vi "SelDataTbl (SubVI).vi"(8 "error in (no error)":errorcluster, 10 "In":dbl[][](array[numeric]), 11 "Enum":T1(ring)) -> (0 "error out":errorcluster, 3 "Out":dbl[][](array[numeric]))   [LabVIEW 2017]
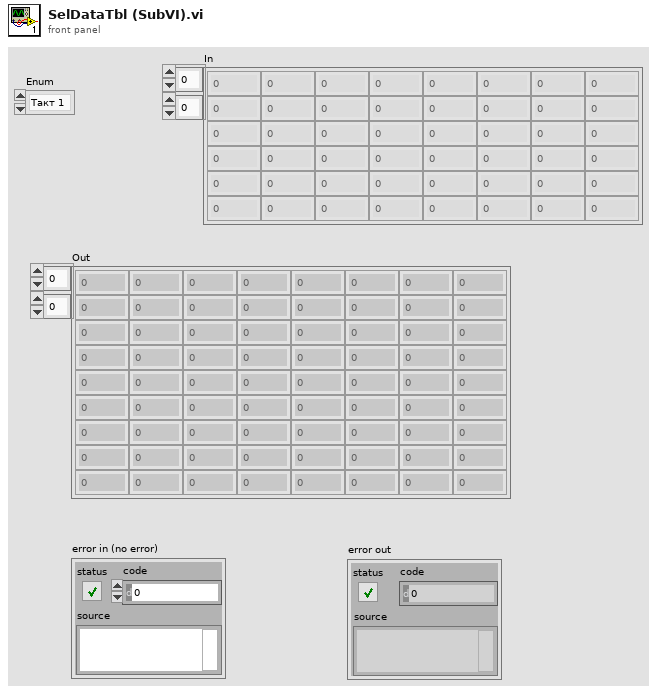
[diagram p1: front panel]
types:
  T1 = enum16{"Такт 1", "Такт 2", "Такт 3", "Такт 4", "Такт 5", "Такт 6", "Такт 7", "Такт 8", "Такт 9", "Такт 10", "Такт 11", "Такт 12", "Такт 13", "Такт 14", "Такт 15", "Такт 16", "Такт 17", "Такт 18", "Такт 19", "Такт 20", "Такт 21", "Такт 22", "Такт 23", "Такт 24", "Такт 25", "Такт 26", "Такт 27", "Такт 28", "Такт 29", "Такт 30", "Такт 31", "Такт 32"}
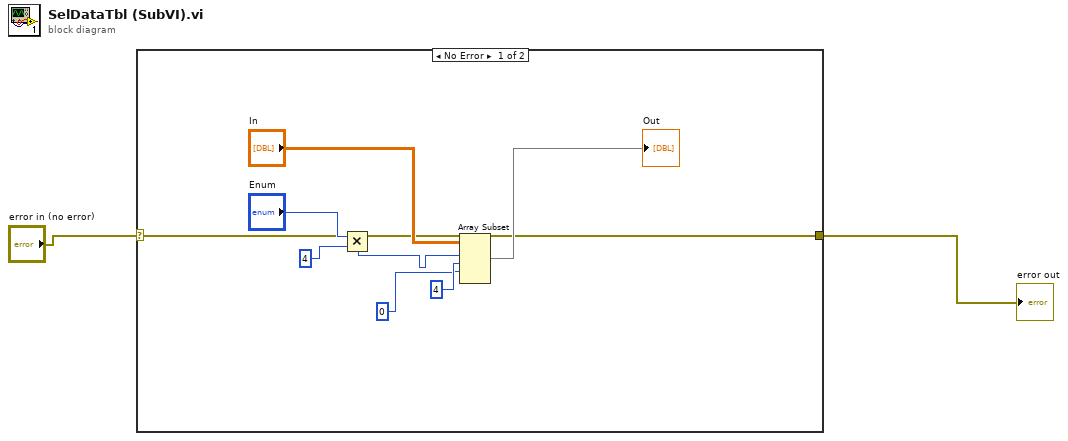
[diagram p0: block diagram]
diagram:
  n1 = case shown="No Error" "error in (no error)" {
    selector: "error in (no error)" -> [w3 w11]
    tunnel: [w3 w11] -> w1
    frame No Error {
      n2 = Multiply(x="Enum", y=4) -> (x*y=w5:i32)
      n3 = Array Subset(array="In", index (row)=w5, length (row)=4 ("length"), index (col)=0 ("index")) -> (→"Out":dbl[][])  [unwired: 1 in]
    }
    frame Error {
    }
  }
  "error out" <- w1
